vi "Set Session Controls.vi"(8 "error in":errorcluster, 10 "Session Controls":refnum<vi>[](array[refnum]), 11 "UI Mode":T1) -> (0 "error out":errorcluster)   [LabVIEW 2026]
doc: "Enables or disables the ATM front-panel controls for one UI Mode, so the main VI needs no property nodes for it. Session Controls is an array of control references in this fixed order: Card Simulator, User Input, Enter, Left Buttons, Right Buttons, Left Menu, Right Menu. Each control is set to Enabled or to Disabled and Grayed Out: Waiting for Card enables only Card Simulator; Card Inserted enables User Input and Enter; Menu Active enables User Input, Enter, both menus and both button clusters; Session Ended disables everything. A missing reference is skipped by LabVIEW with an error.\n\nError behaviour: if error in carries an error, no control is changed and the error is passed to error out."
uses:
  Controls/ATM UI Mode.ctl
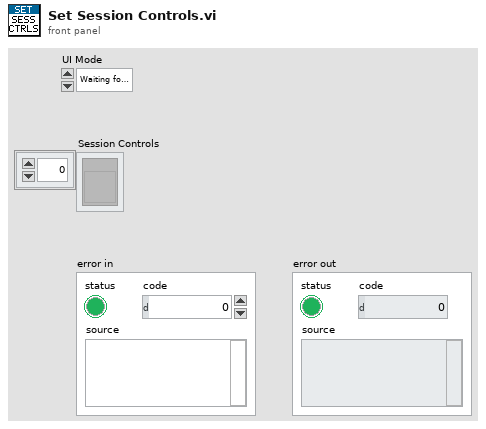
[diagram p1: front panel]
types:
  T1 = typedef "ATM UI Mode.ctl" = enum16{"Waiting for Card", "Card Inserted", "Menu Active", "Session Ended"}
  T2 = enum8{"Enabled", "Disabled", "Disabled and Grayed Out"}[]
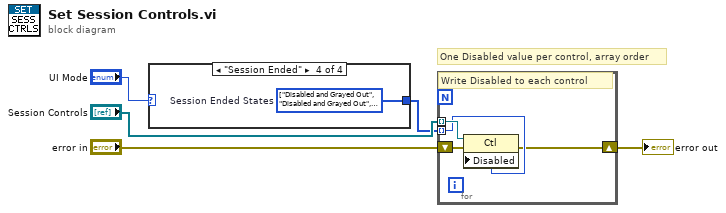
[diagram p0: block diagram]
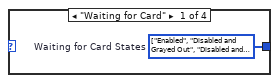
[diagram p2: hidden frame]
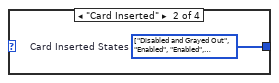
[diagram p3: hidden frame]
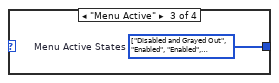
[diagram p4: hidden frame]
diagram:
  # "One Disabled value per control, array order"
  n1 = case shown="\"Session Ended\"" "UI Mode" {
    tunnel: [w6 w7 w8 w9] -> w3
    frame "Waiting for Card" {
      w6 = T2 [enum."Enabled", enum."Disabled and Grayed Out", enum."Disabled and Grayed Out", enum."Disabled and Grayed Out", enum."Disabled and Grayed Out", enum."Disabled and Grayed Out", enum."Disabled and Grayed Out"] items=["Enabled", "Disabled", "Disabled and Grayed Out"]  # Waiting for Card States
    }
    frame "Card Inserted" {
      w7 = T2 [enum."Disabled and Grayed Out", enum."Enabled", enum."Enabled", enum."Disabled and Grayed Out", enum."Disabled and Grayed Out", enum."Disabled and Grayed Out", enum."Disabled and Grayed Out"] items=["Enabled", "Disabled", "Disabled and Grayed Out"]  # Card Inserted States
    }
    frame "Menu Active" {
      w8 = T2 [enum."Disabled and Grayed Out", enum."Enabled", enum."Enabled", enum."Enabled", enum."Enabled", enum."Enabled", enum."Enabled"] items=["Enabled", "Disabled", "Disabled and Grayed Out"]  # Menu Active States
    }
    frame "Session Ended" {
      w9 = T2 [enum."Disabled and Grayed Out", enum."Disabled and Grayed Out", enum."Disabled and Grayed Out", enum."Disabled and Grayed Out", enum."Disabled and Grayed Out", enum."Disabled and Grayed Out", enum."Disabled and Grayed Out"] items=["Enabled", "Disabled", "Disabled and Grayed Out"]  # Session Ended States
    }
  }
  n2 = for {
    tunnel: "Session Controls" -> [w13] mode=indexing
    tunnel: w3 -> [w11] mode=indexing
    shift-right: [w10] -> w1
    shift-left: "error in" -> [w12]
    # "Write Disabled to each control"
    n3 = property class="Ctl"(reference=w13, error in=w12, "Disabled"=w11) -> (error out=w10:errorcluster)  [unwired: 1 out]
  }
  "error out" <- w1
